vi "Scale Double.vi"() -> ()   [LabVIEW 2026]
doc: "Round-12 test-layer subject: y = x * factor. Two doubles in, one out, nothing else - the smallest VI that a generated Caraya test can drive, so what the round measures is the test toolchain and not the subject."
panel:
  out "y":dbl
  in  "factor":dbl
  in  "x":dbl
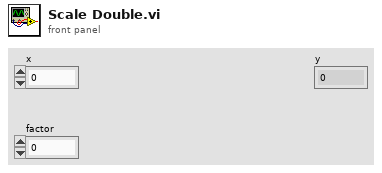
[diagram p1: front panel]
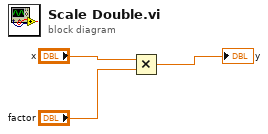
[diagram p0: block diagram]
diagram:
  n1 = Multiply(x="x", y="factor") -> (x*y=→"y":dbl)
